vi "Scaling Parameters.vi"(8 "error in (no error)":errorcluster, 9 "Command Scale":cluster{"Output_Gain":dbl, "Output_Offset":dbl}={"Output_Gain"=1.0, "Output_Offset"=0.0}, 10 "Feedback Scale":cluster{"Input_Gain":dbl, "Input_Offset":dbl}={"Input_Gain"=1.0, "Input_Offset"=0.0}, 11 "Elevator in":refnum<class "Elevator.lvclass">) -> (0 "error out":errorcluster, 3 "Elevator out":refnum<class "Elevator.lvclass">)   [LabVIEW 2021, in "Elevator.lvclass"]
uses:
  Elevator.lvclass
  Elevator.lvclass/Elevator.ctl
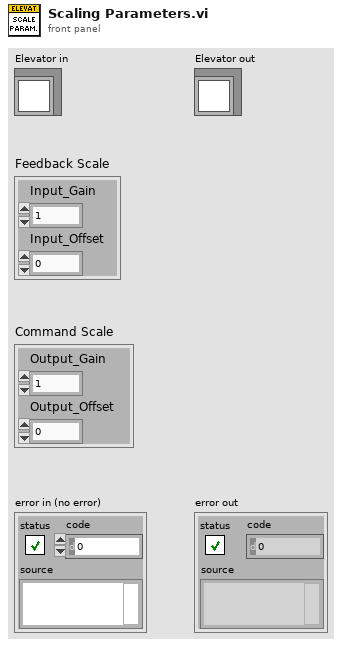
[diagram p1: front panel]
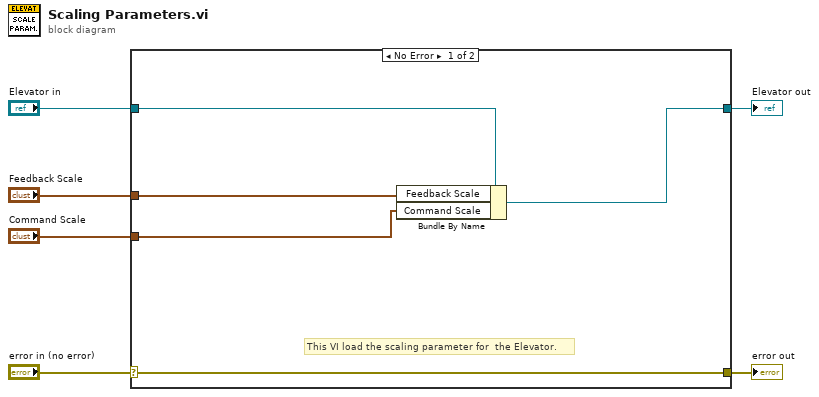
[diagram p0: block diagram]
diagram:
  n1 = case shown="No Error" "error in (no error)" {
    selector: "error in (no error)" -> [w11 w13]
    tunnel: [w11 w13] -> w5
    tunnel: [w9 w12] -> w3
    tunnel: "Elevator in" -> [w10 w12]
    tunnel: "Command Scale" -> [w8 _]
    tunnel: "Feedback Scale" -> [w7 _]
    frame No Error {
      # "This VI load the scaling parameter for  the Elevator."
      n2 = Bundle By Name(cluster=w10, "Feedback Scale"=w7, "Command Scale"=w8) -> (w9:refnum<class "Elevator.lvclass">)
    }
    frame Error {
    }
  }
  "error out" <- w5
  "Elevator out" <- w3
